vi "Save Class.vi"(5 "Clear Before Saving(F)":bool, 7 "PluginPath(T)":bool=TRUE, 8 "error in (no error)":errorcluster, 11 "Channel":refnum<class "Channel.lvclass">) -> (0 "error out":errorcluster, 2 "OK?":bool)   [LabVIEW 2021, in "Channel.lvlib" / "Channel.lvclass"]
uses:
  Channel.lvclass
  <vilib>/Utility/config.llb/Write Key (String).vi
  Configuration_class/Configuration.lvclass
  Channel.lvclass/Channel.ctl
  Channel.lvlib
  <vilib>/Utility/config.llb/NI_LVConfig.lvlib
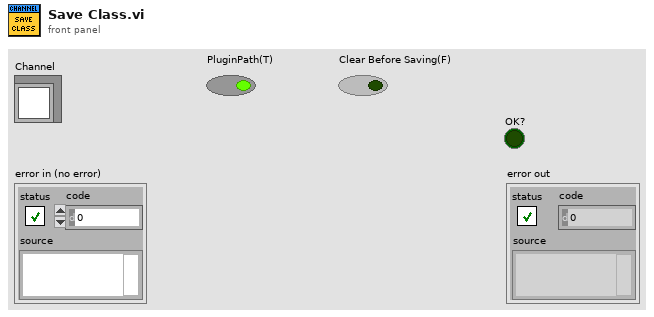
[diagram p1: front panel]
types:
  T1 = typedef "NI_LVConfig.lvlib/Config Data RefNum.ctl" = refnum<k1>
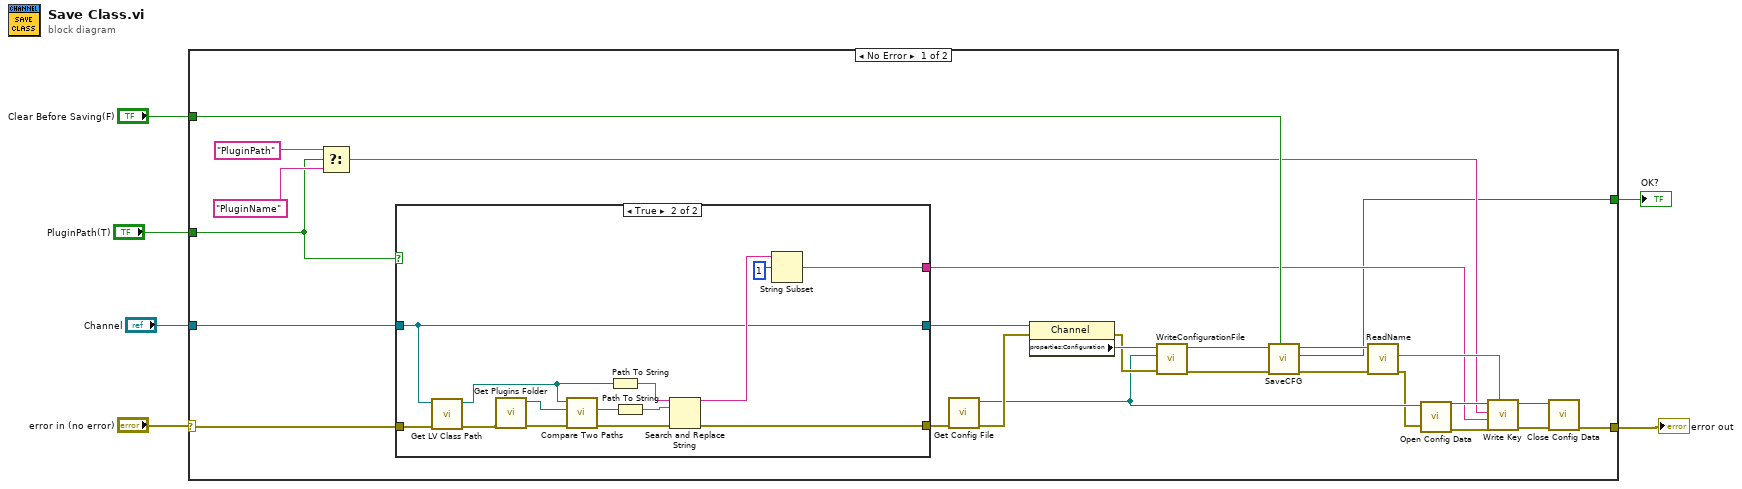
[diagram p0: block diagram]
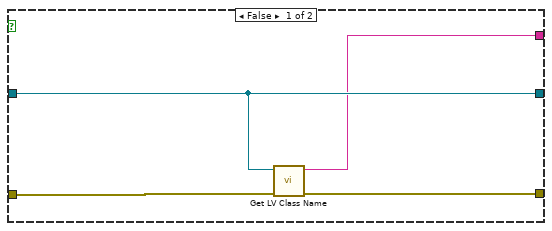
[diagram p2: hidden frame]
diagram:
  n1 = case shown="No Error" "error in (no error)" {
    selector: "error in (no error)" -> [w28 w51]
    tunnel: "Channel" -> [w29 _]
    tunnel: "PluginPath(T)" -> [w30 _]
    tunnel: "Clear Before Saving(F)" -> [w22 _]
    tunnel: [w10 w51] -> w2
    tunnel: [w7 _] -> w1
    frame No Error {
      n2 = Select(t="PluginPath", s=w30, f="PluginName") -> (s? t:f=w13:string)
      n3 = case shown="True" w30 {
        tunnel: w28 -> [w36 w50]
        tunnel: w29 -> [w34 w38]
        tunnel: [w35 w39] -> w27
        tunnel: [w34 w38] -> w26
        tunnel: [w33 w37] -> w8
        frame False {
          n4 = call <vilib>:"Get LV Class Name.vi"("error in (no error)"=w36, "object"=w34) -> ("error out"=w35:errorcluster, "class name"=w33:string)  [unwired: 8 in]
        }
        frame True {
          n5 = call <vilib>:"Get LV Class Path.vi"("error in (no error)"=w50, "object"=w38) -> ("error out"=w49:errorcluster, "class path"=w42:path)  [unwired: 8 in]
          n6 = call "Get Plugins Folder.vi"("error in (no error)"=w49) -> ("error out"=w41:errorcluster, "Plugins Folder"=w43:path)  [unwired: 9 in]
          n7 = call <vilib>:"Compare Two Paths.vi"("error in (no error)"=w41, "Path 2"=w43, "Path 1"=w42) -> ("error out"=w40:errorcluster, "Common Path"=w44:path)  [unwired: 5 in, 2 out]
          n8 = Path To String(path=w42) -> (string=w48:string)
          n9 = Path To String(path=w44) -> (string=w47:string)
          n10 = Search and Replace String(input string=w48, search string=w47, error in=w40) -> (result string=w46:string, error out=w39:errorcluster)  [unwired: 5 in, 2 out]
          n11 = String Subset(string=w46, offset (0)=1) -> (substring=w37:string)  [unwired: 1 in]
        }
      }
      n12 = call "Get Config File.vi"("error in (no error)"=w27) -> ("error out"=w20:errorcluster, "Config File"=w12:path)  [unwired: 9 in]
      n13 = property class="Channel"(reference=w26, error in=w20) -> (error out=w19:errorcluster, "properties:Configuration"=w25:refnum<class "Configuration.lvclass">)  [unwired: 1 out]
      n14 = call "WriteConfigurationFile.vi"("error in (no error)"=w19, "Configuration File"=w12, "object in"=w25) -> ("error out"=w18:errorcluster, "object out"=w24:refnum<class "Configuration.lvclass">)  [unwired: 7 in]
      n15 = call-dynamic "SaveCFG.vi"("Clear Before Saving(F)"=w22, "error in (no error)"=w18, "object in"=w24) -> ("error out"=w21:errorcluster, "OK?"=w7:bool, "object out"=w23:refnum<class "Configuration.lvclass">)  [unwired: 6 in]
      n16 = call-dynamic "ReadName.vi"("error in (no error)"=w21, "object in"=w23) -> ("error out"=w11:errorcluster, "Name"=w14:string)  [unwired: 7 in, 1 out]
      n17 = call <vilib>:"Open Config Data.vi"("error in (no error)"=w11, "configuration file path"=w12) -> ("error out"=w9:errorcluster, "refnum"=w15:T1)  [unwired: 7 in, 1 out]
      n18 = call-poly <vilib>:"Write Key.vi"("section"=w14, "error in (no error)"=w9, "value"=w8, "key"=w13, "refnum"=w15) -> ("error out"=w17:errorcluster, "refnum out"=w16:T1)  [unwired: 4 in, 1 out]
      n19 = call <vilib>:"Close Config Data.vi"("error in (no error)"=w17, "refnum"=w16) -> ("error out"=w10:errorcluster)  [unwired: 8 in, 1 out]
    }
    frame Error {
    }
  }
  "error out" <- w2
  "OK?" <- w1
